vi "REST_Call_Paced.vi"(7 "method":T2, 8 "error in (no error)":errorcluster, 9 "body":string, 10 "url":string, 11 "client handle":T1) -> (0 "error out":errorcluster, 1 "response":string, 2 "status":i32, 3 "client handle out":T1)   [LabVIEW 2021, in "CANsub_Common.lvlib"]
doc: "REST_Call followed by a pause of 20 ms. For groups of calls (channel open), so that the device does not get REST calls with no pause. Setup/teardown only: do not call in a periodic loop (allocates, may block)."
uses:
  CANsub_Common.lvlib
  <vilib>/httpClient/ClientHandle.ctl
  <vilib>/httpClient/LabVIEWHTTPClient.lvlib
  Typedefs/HTTP_Method.ctl
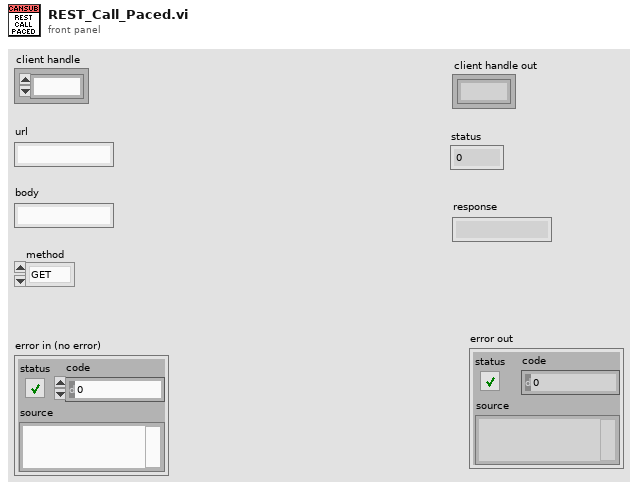
[diagram p1: front panel]
types:
  T1 = typedef "LabVIEWHTTPClient.lvlib/ClientHandle.ctl" = refnum<k1>
  T2 = typedef "CANsub_Common.lvlib/HTTP_Method.ctl" = enum16{"GET", "PUT", "POST", "DELETE"}
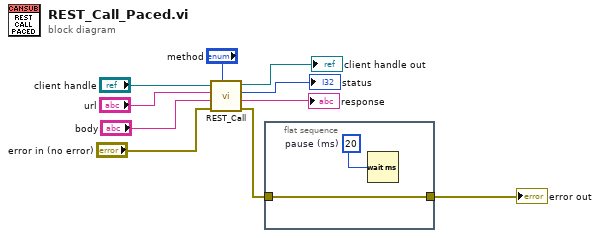
[diagram p0: block diagram]
diagram:
  n1 = call "REST_Call.vi"("method"="method", "error in (no error)"="error in (no error)", "body"="body", "url"="url", "client handle"="client handle") -> ("error out"=w2:errorcluster, "response"=→"response":string, "status"=→"status":i32, "client handle out"=→"client handle out":T1)  [unwired: 3 in]
  n2 = flat-sequence {
    tunnel: [w12] -> w1
    tunnel: w2 -> [w12]
    frame #0 {
      w11 = u32 20  # pause (ms)
      n3 = Wait (ms)(milliseconds to wait=w11) -> ()  [unwired: 1 out]
    }
  }
  "error out" <- w1
